vi "Acqui Tout MODBUS.vi"(3 "error in (no error)":errorcluster caption="entrée d'erreur (pas d'erreur)", 5 "Adresse régulateur":u8, 6 "Port COM":u16(ring) items=["COM1"]) -> (0 "error out":errorcluster caption="entrée d'erreur (pas d'erreur)", 1 "Al sur mesure":string[](array[string]), 2 "data reg":string[](array[string]))   [LabVIEW 2022 SP3]
uses:
  Variables globales/Variables glob EUROTHERM.vi
  Variables globales/Variable glob generale.vi
panel:
  out "Al haute mesure":string
  out "Al basse mesure":string
  out "Al haute sécu":string
  out "Al basse sécu":string
  out "Sécu":string
  out "Consigne":string
  out "Mesure":string
  out "Puissance":string
  # "acquisitions données modbus"
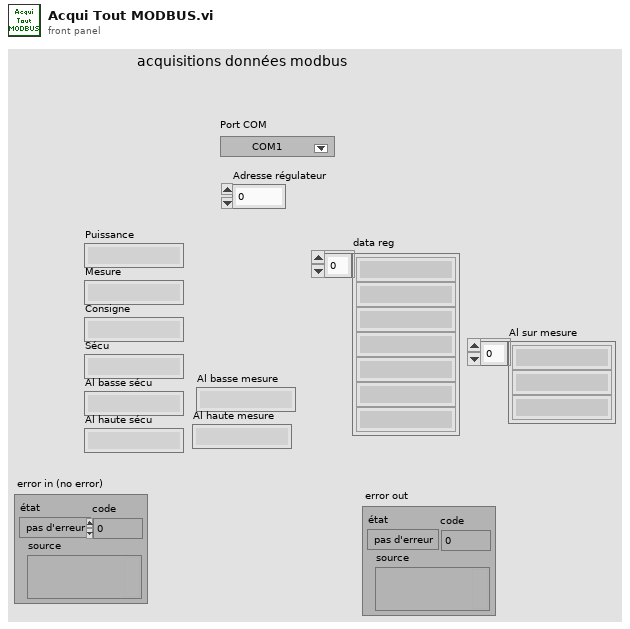
[diagram p1: front panel]
types:
  T1 = typedef "Semaphore RefNum" = refnum<k1>
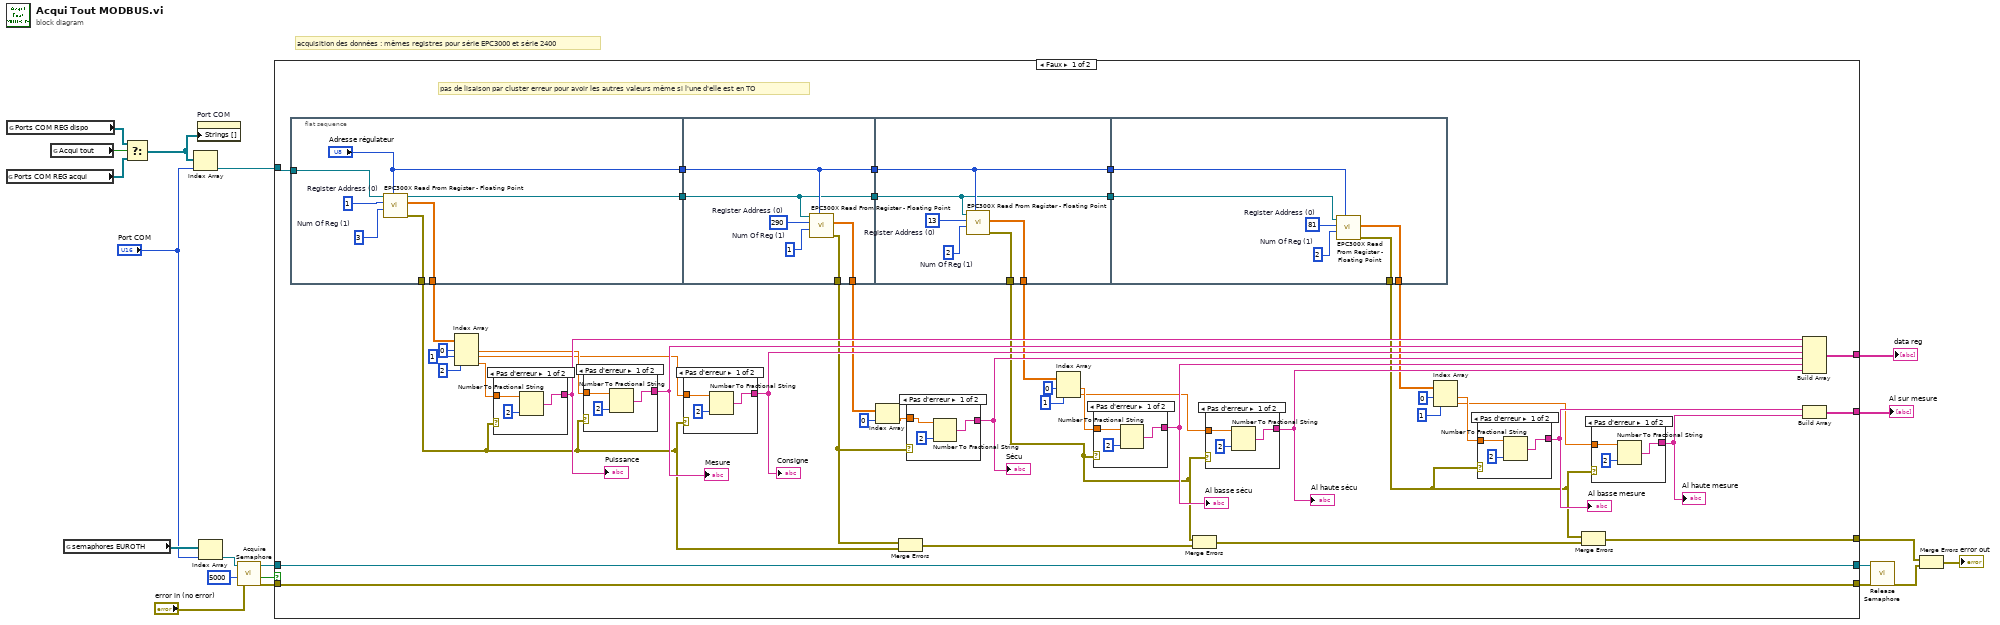
[diagram p0: block diagram]
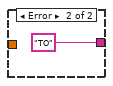
[diagram p2: hidden frame]
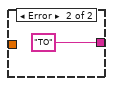
[diagram p3: hidden frame]
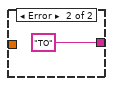
[diagram p4: hidden frame]
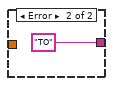
[diagram p5: hidden frame]
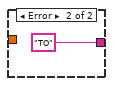
[diagram p6: hidden frame]
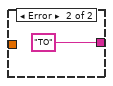
[diagram p7: hidden frame]
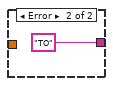
[diagram p8: hidden frame]
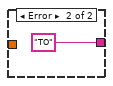
[diagram p9: hidden frame]
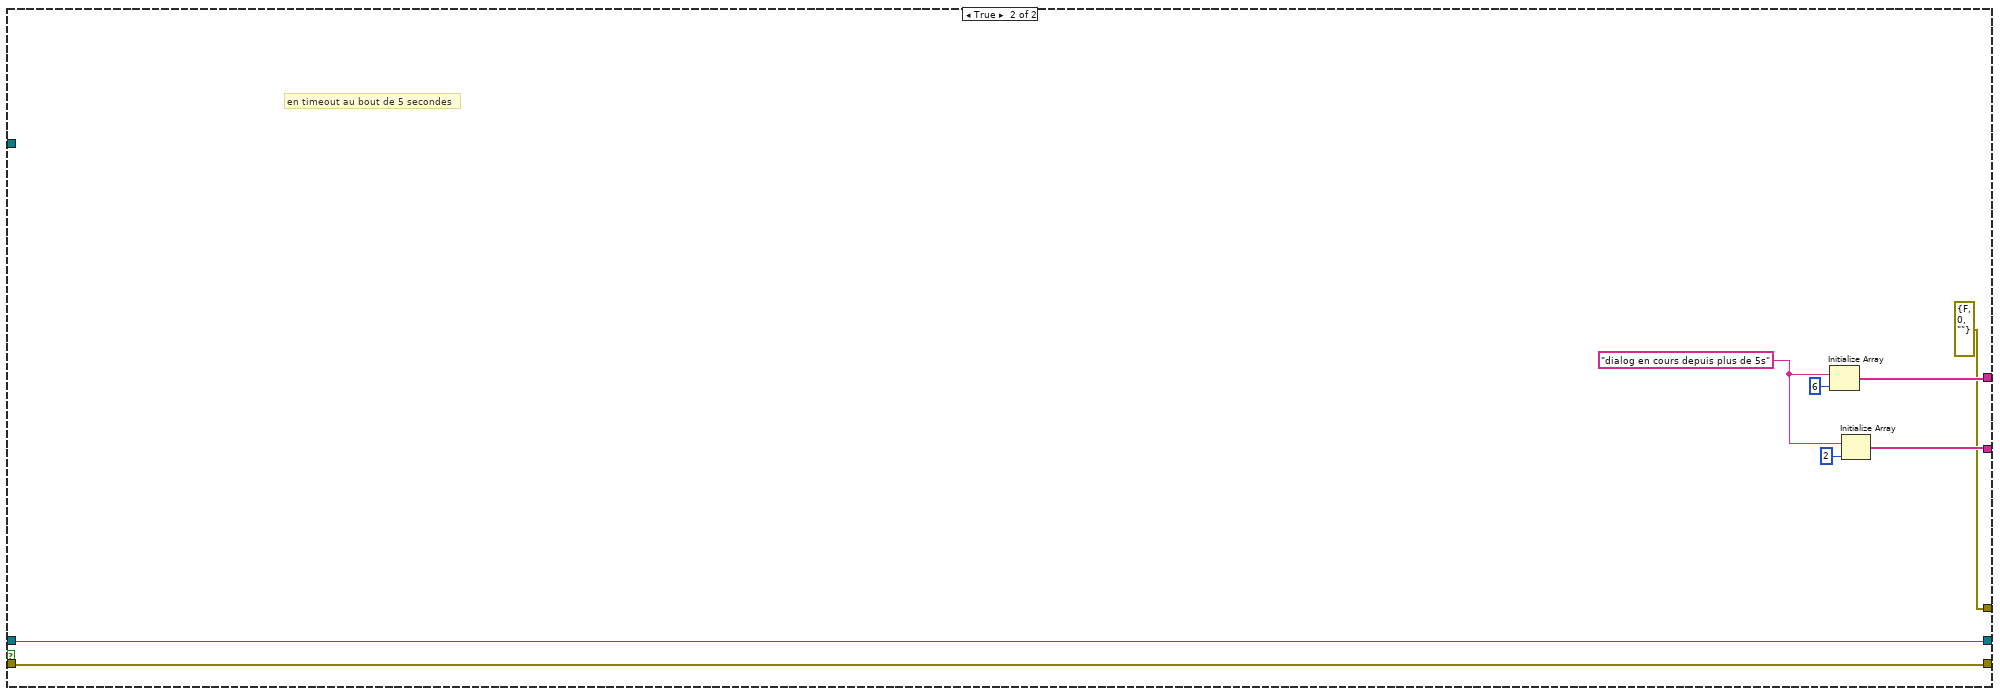
[diagram p10: hidden frame]
diagram:
  # "acquisition des données : mêmes registres pour série EPC3000 et série 2400"
  n1 = global read "Variables glob EUROTHERM.vi" "Ports COM REG acqui"() -> (w6:refnum<visa-resource-name>[])
  n2 = global read "Variables glob EUROTHERM.vi" "Ports COM REG dispo"() -> (w7:refnum<visa-resource-name>[])
  n3 = global read "Variable glob generale.vi" "Acqui tout"() -> (w8:bool)
  n4 = global read "Variables glob EUROTHERM.vi" "semaphores EUROTH"() -> (w12:T1[])
  n5 = Select(t=w7, s=w8, f=w6) -> (s? t:f=w5:refnum<visa-resource-name>[])
  n6 = Index Array(array=w5, index="Port COM") -> (element=w10:refnum<visa-resource-name>)
  n7 = property on="Port COM" class="MDér (strict)"("Strings []"=w5) -> ()  [unwired: 2 in, 2 out]
  n8 = Index Array(array=w12, index="Port COM") -> (element=w11:T1)
  n9 = call <vilib>:"Acquire Semaphore.vi"("error in (no error)"="error in (no error)", "ms timeout (-1)"=5000, "semaphore"=w11) -> ("error out"=w19:errorcluster, "timed out"=w20:bool, "semaphore out"=w17:T1)  [unwired: 2 in]
  n10 = case shown="Faux" w20 {
    tunnel: [w64 w128] -> w13
    tunnel: w19 -> [w66 w130]
    tunnel: [w66 w130] -> w18
    tunnel: w17 -> [w65 w131]
    tunnel: [w65 w131] -> w16
    tunnel: w10 -> [w53 _]
    tunnel: [w63 w125] -> w4
    tunnel: [w21 errorcluster {"status"=FALSE, "code"=0, "source"=""} ("error out")] -> w3
    frame False {
      # "pas de lisaison par cluster erreur pour avoir les autres valeurs même si l'une d'elle est en TO"
      n11 = flat-sequence {
        tunnel: [w72] -> w56
        tunnel: w53 -> [w68]
        tunnel: [w67] -> w26
        tunnel: [w73] -> w36
        tunnel: ["Adresse régulateur"] -> w35
        tunnel: w36 -> [w74]
        tunnel: w35 -> [w75]
        tunnel: [w77] -> w34
        tunnel: [w76] -> w27
        tunnel: [w75] -> w33
        tunnel: [w74] -> w32
        tunnel: w33 -> [w81]
        tunnel: w32 -> [w80]
        tunnel: [w83] -> w31
        tunnel: [w82] -> w25
        tunnel: [w81] -> w30
        tunnel: [w80] -> w29
        tunnel: w30 -> [w89]
        tunnel: w29 -> [w88]
        tunnel: [w87] -> w28
        tunnel: [w86] -> w23
        frame #0 {
          w71 = u16 1  # Register Address (0)
          w70 = u16 3  # Num Of Reg (1)
          n12 = call "EPC300X Read From Register - Floating Point.vi"("Unit Address (1)"="Adresse régulateur", "Num Of Reg (1)"=w70, "Register Address (0)"=w71, "VISA session"=w68) -> ("error out"=w67:errorcluster, "Data (SGL)"=w72:sgl[], "dup VISA session"=w73:refnum<visa-resource-name>)  [unwired: 2 in, 3 out]
        }
        frame #1 {
          w78 = u16 290  # Register Address (0)
          w79 = u16 1  # Num Of Reg (1)
          n13 = call "EPC300X Read From Register - Floating Point.vi"("Unit Address (1)"=w75, "Num Of Reg (1)"=w79, "Register Address (0)"=w78, "VISA session"=w74) -> ("error out"=w76:errorcluster, "Data (SGL)"=w77:sgl[])  [unwired: 2 in, 4 out]
        }
        frame #2 {
          w84 = u16 2  # Num Of Reg (1)
          w85 = u16 13  # Register Address (0)
          n14 = call "EPC300X Read From Register - Floating Point.vi"("Unit Address (1)"=w81, "Num Of Reg (1)"=w84, "Register Address (0)"=w85, "VISA session"=w80) -> ("error out"=w82:errorcluster, "Data (SGL)"=w83:sgl[])  [unwired: 2 in, 4 out]
        }
        frame #3 {
          w91 = u16 2  # Num Of Reg (1)
          w90 = u16 81  # Register Address (0)
          n15 = call "EPC300X Read From Register - Floating Point.vi"("Unit Address (1)"=w89, "Num Of Reg (1)"=w91, "Register Address (0)"=w90, "VISA session"=w88) -> ("error out"=w86:errorcluster, "Data (SGL)"=w87:sgl[])  [unwired: 2 in, 4 out]
        }
      }
      n16 = Index Array(array=w56, index #1=0 ("indice"), index #2=1 ("indice"), index #3=2 ("indice")) -> (element #1=w50:sgl, element #2=w48:sgl, element #3=w52:sgl)
      n17 = case shown="Pas d'erreur" w26 {
        tunnel: w52 -> [w121 _]
        tunnel: [w120 "TO"] -> w51
        frame No Error {
          n18 = Number To Fractional String(number=w121, precision (6)=i16 2 ("précision (6)")) -> (F-format string=w120:string)  [unwired: 2 in]
        }
        frame Error {
        }
      }
      "Puissance" <- w51
      n19 = case shown="Pas d'erreur" w26 {
        tunnel: w50 -> [w117 _]
        tunnel: [w116 "TO"] -> w49
        frame No Error {
          n20 = Number To Fractional String(number=w117, precision (6)=i16 2 ("précision (6)")) -> (F-format string=w116:string)  [unwired: 2 in]
        }
        frame Error {
        }
      }
      "Mesure" <- w49
      n21 = case shown="Pas d'erreur" w26 {
        tunnel: w48 -> [w113 _]
        tunnel: [w112 "TO"] -> w47
        frame No Error {
          n22 = Number To Fractional String(number=w113, precision (6)=i16 2 ("précision (6)")) -> (F-format string=w112:string)  [unwired: 2 in]
        }
        frame Error {
        }
      }
      "Consigne" <- w47
      n23 = Index Array(array=w34, index=0 ("indice")) -> (element=w46:sgl)
      n24 = Merge Errors(w27, w26) -> (w24:errorcluster)
      n25 = case shown="Pas d'erreur" w27 {
        tunnel: [w109 "TO"] -> w45
        tunnel: w46 -> [w108 _]
        frame No Error {
          n26 = Number To Fractional String(number=w108, precision (6)=i16 2 ("précision (6)")) -> (F-format string=w109:string)  [unwired: 2 in]
        }
        frame Error {
        }
      }
      "Sécu" <- w45
      n27 = Index Array(array=w31, index #1=0 ("index"), index #2=1 ("indice")) -> (element #1=w44:sgl, element #2=w42:sgl)
      n28 = case shown="Pas d'erreur" w25 {
        tunnel: w44 -> [w105 _]
        tunnel: [w104 "TO"] -> w43
        frame No Error {
          n29 = Number To Fractional String(number=w105, precision (6)=i16 2 ("précision (6)")) -> (F-format string=w104:string)  [unwired: 2 in]
        }
        frame Error {
        }
      }
      "Al basse sécu" <- w43
      n30 = Merge Errors(w25, w24) -> (w22:errorcluster)
      n31 = case shown="Pas d'erreur" w25 {
        tunnel: w42 -> [w101 _]
        tunnel: [w100 "TO"] -> w41
        frame No Error {
          n32 = Number To Fractional String(number=w101, precision (6)=i16 2 ("précision (6)")) -> (F-format string=w100:string)  [unwired: 2 in]
        }
        frame Error {
        }
      }
      "Al haute sécu" <- w41
      n33 = Index Array(array=w28, index #1=0 ("index"), index #2=1 ("indice")) -> (element #1=w40:sgl, element #2=w38:sgl)
      n34 = case shown="Pas d'erreur" w23 {
        tunnel: w40 -> [w97 _]
        tunnel: [w96 "TO"] -> w39
        frame No Error {
          n35 = Number To Fractional String(number=w97, precision (6)=i16 2 ("précision (6)")) -> (F-format string=w96:string)  [unwired: 2 in]
        }
        frame Error {
        }
      }
      "Al basse mesure" <- w39
      n36 = Merge Errors(w23, w22) -> (w21:errorcluster)
      n37 = case shown="Pas d'erreur" w23 {
        tunnel: w38 -> [w93 _]
        tunnel: [w92 "TO"] -> w37
        frame No Error {
          n38 = Number To Fractional String(number=w93, precision (6)=i16 2 ("précision (6)")) -> (F-format string=w92:string)  [unwired: 2 in]
        }
        frame Error {
        }
      }
      "Al haute mesure" <- w37
      n39 = Build Array(w51, w49, w47, w45, w43, w41) -> (w64:string[])
      n40 = Build Array(w39, w37) -> (w63:string[])
    }
    frame True {
      w126 = "dialog en cours depuis plus de 5s"
      # "en timeout au bout de 5 secondes"
      n41 = Initialize Array(w126, 6 ("taille de la dimension")) -> (w128:string[])
      n42 = Initialize Array(w126, 2 ("taille de la dimension")) -> (w125:string[])
    }
  }
  "data reg" <- w13
  "Al sur mesure" <- w4
  n43 = call <vilib>:"Release Semaphore.vi"("error in (no error)"=w18, "semaphore"=w16) -> ("error out"=w2:errorcluster)  [unwired: 4 in, 1 out]
  n44 = Merge Errors(w3, w2) -> (→"error out":errorcluster)
